vi "Get Rx Hardware Channel Data.vi"(8 "error in":errorcluster, 11 "custom device ref in":T2 format="%.0x") -> (0 "error out":errorcluster, 1 "Rx hardware channel data":T3[](array[typedef]) {"labels settings for RT"."Label Timestamp Channel Data Reference" format="%.0x"; "labels settings for RT"."Word Initial Raw Value" format="%032.0f"; "labels settings for RT"."Label Disable/Trigger Channel Reference" format="%.0x"; "labels settings for RT"."parameter driver data"."Tx parameter refs" format="%.0x"; "labels settings for RT"."SDI" format="%02b"; "labels settings for RT"."label" format="%.0o"}, 2 "incoming channels":T2[](array[typedef]) format="%.0x", 3 "custom device ref out":T2 format="%.0x", 4 "channel data offsets":T1)   [LabVIEW 2020]
uses:
  <vilib>/NI VeriStand/Custom Device API/Custom Device Item Ref.ctl
  <vilib>/NI VeriStand/Custom Device API/Custom Device API.lvlib
  Label.ctl
  <vilib>/NI/NI VeriStand Encoding and Decoding/Encoding.ctl
  <vilib>/NI/NI VeriStand Encoding and Decoding/Encoding and Decoding.lvlib
  <vilib>/NI VeriStand/Custom Device API/Data Reference.ctl
  RT Parameters.ctl
  RT Label Settings.ctl
  RT Hardware Channel Settings.ctl
  Transfer Type.ctl
  Parameter Definition.ctl
  Scripting/Ballard/Ballard ARINC 429 Scripting.lvlib
  Scripting/ARINC 429/ARINC 429 Scripting.lvlib
  Rx Channel Data Offsets.ctl
  Engine/Custom Device/Custom Device.lvlib
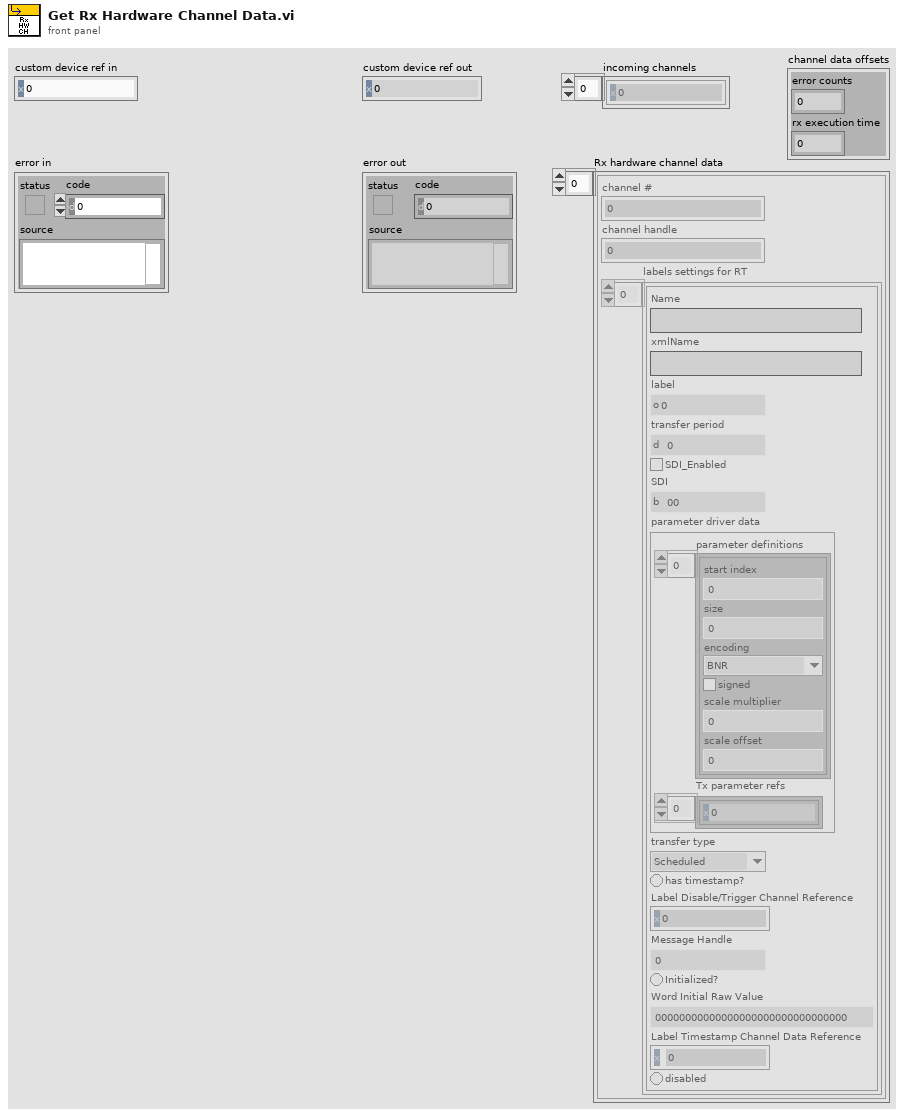
[diagram p1: front panel]
types:
  T1 = typedef "Rx Channel Data Offsets.ctl" = cluster{"error counts":u32, "rx execution time":i64}
  T2 = typedef "Custom Device API.lvlib/Custom Device Item Ref.ctl" = u64
  T3 = typedef "RT Hardware Channel Settings.ctl" = cluster{"channel #":u16, "channel handle":u64, "labels settings for RT":T4[]}
  T4 = typedef "RT Label Settings.ctl" = cluster{"Name":string, "xmlName":string, "label":T5, "transfer period":u32, "SDI_Enabled":bool, "SDI":u8, "parameter driver data":T6, "transfer type":T9, "has timestamp?":bool, "Label Disable/Trigger Channel Reference":T2, "Message Handle":u64, "Initialized?":bool, "Word Initial Raw Value":u32, "Label Timestamp Channel Data Reference":T10, "disabled":bool}
  T5 = typedef "Label.ctl" = u8
  T6 = typedef "RT Parameters.ctl" = cluster{"parameter definitions":T7[], "Tx parameter refs":T2[]}
  T7 = typedef "Parameter Definition.ctl" = cluster{"start index":i32, "size":i32, "encoding":T8, "signed":bool, "scale multiplier":dbl, "scale offset":dbl}
  T8 = typedef "Encoding and Decoding.lvlib/Encoding.ctl" = enum16{"BNR", "BCD", "Discrete"}
  T9 = typedef "Transfer Type.ctl" = enum16{"Scheduled", "Acyclic", "Block", "Strobe"}
  T10 = typedef "Custom Device API.lvlib/Data Reference.ctl" = i32
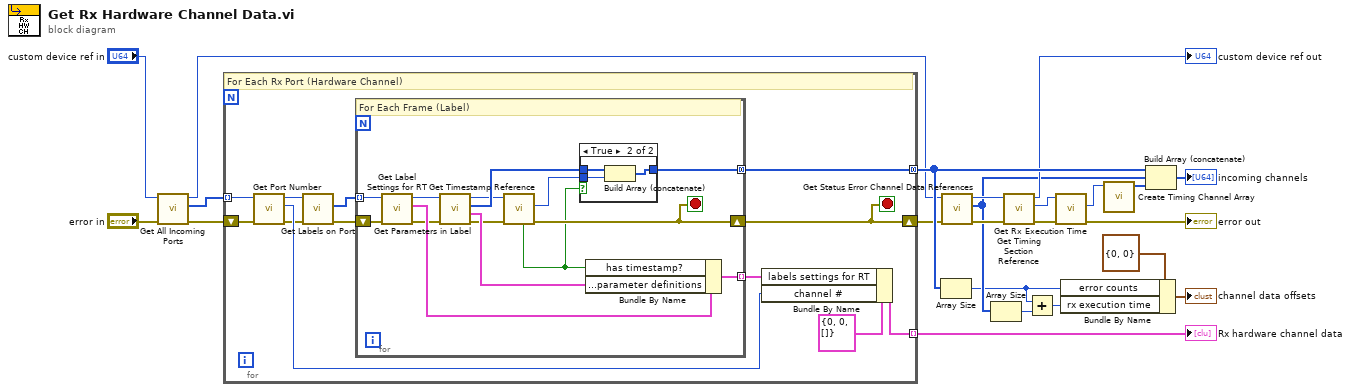
[diagram p0: block diagram]
diagram:
  n1 = call "Get All Incoming Ports.vi"("error in"="error in", "Ballard ARINC 429 custom device in"="custom device ref in") -> ("error out"=w20:errorcluster, "incoming ports"=w19:T2[], "Ballard ARINC 429 custom device out"=w9:T2)  [unwired: 7 in]
  n2 = for {
    shift-right: [w34] -> w10
    shift-left: w20 -> [w29]
    tunnel: w19 -> [w30] mode=indexing
    tunnel: [w33] -> w21 mode=indexing
    tunnel: [w23] -> w15 mode=concatenating
    stop <- w34 stop-if-true
    # "For Each Rx Port (Hardware Channel)"
    n3 = call "Get Port Number.vi"("error in"=w29, "port ref in"=w30) -> ("error out"=w26:errorcluster, "port number"=w28:u16, "port ref out"=w27:T2)  [unwired: 6 in, 1 out]
    n4 = call "Get Labels on Port.vi"("error in"=w26, "port in"=w27) -> ("error out"=w24:errorcluster, "labels"=w25:T2[])  [unwired: 6 in, 2 out]
    n5 = for {
      tunnel: w25 -> [w48] mode=indexing
      shift-right: [w36] -> w34
      shift-left: w24 -> [w47]
      tunnel: [w44] -> w32 mode=indexing
      tunnel: [w41] -> w23 mode=concatenating
      stop <- w36 stop-if-true
      # "For Each Frame (Label)"
      n6 = call "Get Label Settings for RT.vi"("error in"=w47, "label ref in"=w48) -> ("error out"=w39:errorcluster, "label settings for RT"=w46:T4, "label ref out"=w40:T2)  [unwired: 7 in]
      n7 = call "Get Parameters in Label.vi"("error in"=w39, "label in"=w40) -> ("error out"=w37:errorcluster, "parameter definitions"=w45:T7[], "parameters"=w43:T2[], "label out"=w38:T2)  [unwired: 6 in]
      n8 = call "Get Timestamp Reference.vi"("error in"=w37, "label ref in"=w38) -> ("error out"=w36:errorcluster, "timestamp channel reference"=w42:T2, "timestamp channel found?"=w35:bool)  [unwired: 6 in, 1 out]
      n9 = case shown="True" w35 {
        tunnel: w43 -> [w49 w52]
        tunnel: w42 -> [_ w51]
        tunnel: [w49 w50] -> w41
        frame False {
        }
        frame True {
          n10 = Build Array (concatenate)(w52, w51) -> (w50:T2[])
        }
      }
      n11 = Bundle By Name(cluster=w46, "has timestamp?"=w35, "parameter driver data.parameter definitions"=w45) -> (w44:T4)
    }
    n12 = Bundle By Name(cluster=T3 {"channel #"=0, "channel handle"=0, "labels settings for RT"=[]} ("RT hardware channel"), "labels settings for RT"=w32, "channel #"=w28) -> (w33:T3)
  }
  "Rx hardware channel data" <- w21
  n13 = Array Size(array=w15) -> (size(s)=w3:i32)
  n14 = call "Get Status Error Channel Data References.vi"("error in"=w10, "custom device ref in"=w9) -> ("error out"=→"error out":errorcluster, "status channel data references"=w6:T2[], "custom device ref out"=w12:T2)  [unwired: 7 in]
  n15 = Array Size(array=w6) -> (size(s)=w5:i32)
  n16 = call "Get Timing Section Reference.vi"("Ballard ARINC 429 ref"=w12) -> ("error out"=w14:errorcluster, "timing section ref"=w13:T2, "Ballard ARINC 429 ref out"=→"custom device ref out":T2)  [unwired: 7 in, 1 out]
  n17 = Add(x=w3, y=w5) -> (x+y=w4:i32)
  n18 = call "Get Rx Execution Time.vi"("error in"=w14, "timing section in"=w13) -> ("rx execution time ref"=w2:T2)  [unwired: 7 in, 2 out]
  n19 = Bundle By Name(cluster=T1 {"error counts"=0, "rx execution time"=0} ("channel data offsets"), "error counts"=w3, "rx execution time"=w4) -> (→"channel data offsets":T1)
  n20 = call "Create Timing Channel Array.vi"("timing channel ref"=w2) -> ("timing channel ref array"=w1:T2[])  [unwired: 9 in, 1 out]
  n21 = Build Array (concatenate)(w15, w6, w1) -> (→"incoming channels":T2[])
